vi "labview-quick-csv.vi"   [LabVIEW 2020]
uses:
  Nominal Client/Nominal Client.lvclass/Nominal Client.ctl
  User/User.lvclass
  Nominal Client/Nominal Client.lvclass
  nominal types/workspace/workspace.lvclass
  submodules/reqwest-labview/lv-src/reqwest/reqwest.lvclass
  e79185ee-863a-4b48-b269-365b27d9e424.vi
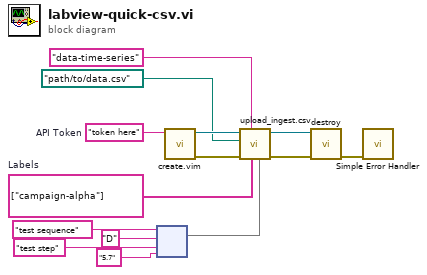
[diagram p0: block diagram]
diagram:
  w2 = string[] ["campaign-alpha"]  # Labels
  w13 = "token here"  # API Token
  n1 = node("test sequence", "D", "test step", "5.7") -> (w1:map{string, string})
  n2 = call "create.vim"("API Token (string or path)"=w13) -> ("error out"=w6:errorcluster, "Nominal Client"=w8:refnum<class "Nominal Client.lvclass">)  [unwired: 8 in, 1 out]
  n3 = call "upload_ingest.csv.vi"("Properties"=w1, "Labels"=w2, "Timestamp SeriesName"="data-time-series", "error in"=w6, "File Path"=path "path/to/data.csv", "Nominal Client in"=w8) -> ("error out"=w5:errorcluster, "Nominal Client out"=w7:refnum<class "Nominal Client.lvclass">)  [unwired: 3 in, 1 out]
  n4 = call "destroy.vi"("error in"=w5, "Nominal Client"=w7) -> ("error out"=w14:errorcluster)  [unwired: 9 in]
  n5 = call <vilib>:"Simple Error Handler.vi"("error in (no error)"=w14) -> ()  [unwired: 4 in, 5 out]
